vi "Measure.vi"(8 "error in (no error)":errorcluster, 9 "measurement configuration":variant, 10 "measure call context in":refnum<class "Measure Call Context.lvclass">, 11 "measurement plugin in":refnum<class "CAN-LIN Raw Bus Capture.lvclass">) -> (0 "error out":errorcluster, 1 "measurement results":variant, 2 "measure call context out":refnum<class "Measure Call Context.lvclass">, 3 "measurement plugin out":refnum<class "CAN-LIN Raw Bus Capture.lvclass">)   [LabVIEW 2025, in "CAN-LIN Raw Bus Capture.lvclass"]
uses:
  CAN-LIN Raw Bus Capture.lvclass
  CAN-LIN Raw Bus Capture.lvclass/CAN-LIN Raw Bus Capture.ctl
  Measurement Configuration.ctl
  CAN-LIN Raw Bus Capture UI/Toggle.ctl
  OOB gRPC Server/OOB gRPC Server.lvlib
  OOB Data Transfer/OOB Data Transfer.lvlib
  <vilib>/Plug-In SDKs/Measurements/Measure Call Context/Measure Call Context.lvclass
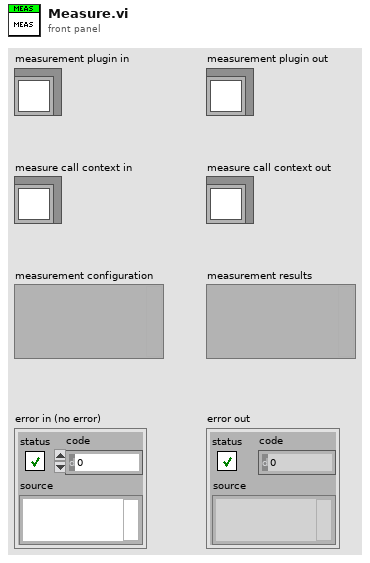
[diagram p1: front panel]
types:
  T1 = typedef "CAN-LIN Raw Bus Capture.lvclass/Measurement Configuration.ctl" = cluster{"Termination CAN":T2, "FD Baudrate":u32, "Baudrate":u32, "FD ISO Mode":enum32{"ISO", "Legacy ISO", "Non-ISO"}, "IO Mode":enum32{"CAN", "CAN FD", "CAN FD + BRS"}, "Termination LIN":T2, "Can Interface":string, "Lin Interface":string, "Bus Type":string, "INTERFACE NAME CAN":refnum<k21>, "INTERFACE NAME LIN":refnum<k21>}
  T2 = typedef "Toggle.ctl" = bool
  T3 = typedef "CAN-LIN Raw Bus Capture.lvclass/Measurement Results.ctl" = cluster{"Message Buffer":string[][], "Status":string, "OOB gRPC Port":i32, "Connection":bool, "Error (Logic)":string, "Buffer Size":i32}
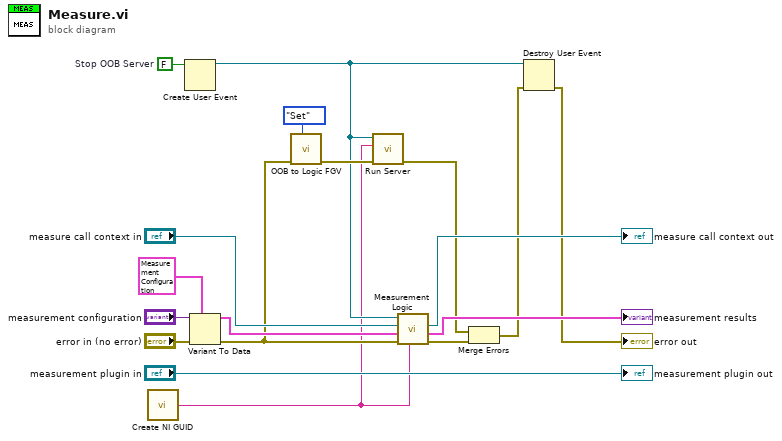
[diagram p0: block diagram]
diagram:
  w10 = FALSE  # Stop OOB Server
  n1 = call <vilib>:"Create NI GUID.vi"() -> ("NI GUID"=w1:string)
  n2 = Create User Event(user event datatype=w10) -> (user event=w6:refnum<user-event>)  [unwired: 1 in, 1 out]
  n3 = Variant To Data(error in="error in (no error)", type=T1 {"Termination CAN"=FALSE, "FD Baudrate"=1, "Baudrate"=32, "FD ISO Mode"=enum."Non-ISO", "IO Mode"=enum."CAN FD + BRS", "Termination LIN"=FALSE, "Can Interface"="", "Lin Interface"="", "Bus Type"="", "INTERFACE NAME CAN"="", "INTERFACE NAME LIN"=""} ("measurement configuration"), Variant="measurement configuration") -> (data=w11:T1, error out=w8:errorcluster)
  n4 = call "OOB to Logic FGV.vi"("Op (Get)"=enum16{"Get", "Set"}."Set", "error in (no error)"=w8) -> ("error out"=w7:errorcluster)  [unwired: 8 in, 1 out]
  n5 = call "Run Server.vi"("error in (no error)"=w7, "NI GUID"=w1, "Stop OOB Server UE"=w6) -> ("error out"=w4:errorcluster)  [unwired: 8 in]
  n6 = call "Measurement Logic.vi"("NI GUID"=w1, "error in"=w8, "measurement configuration"=w11, "measure call context in"="measure call context in", "Stop OOB Server UE"=w6) -> ("error out"=w5:errorcluster, "measurement results"=→"measurement results":T3, "measure call context out"=→"measure call context out":refnum<class "Measure Call Context.lvclass">)  [unwired: 4 in]
  n7 = Merge Errors(w4, w5) -> (w3:errorcluster)
  n8 = Destroy User Event(user event=w6, error in=w3) -> (error out=→"error out":errorcluster)
  "measurement plugin out" <- "measurement plugin in"
